vi "VIH HelpGen - Write HTML File - Menu - VI Table.vi"(4 "Show Item Icons":bool, 5 "HTML Folder":path, 6 "Items":T1, 7 "Image Folder":path, 8 "error in":errorcluster, 9 "Table Templates":T2, 10 "HTML in":string, 11 "Menu Path":path) -> (0 "error out":errorcluster, 2 "HTML out":string, 3 "dup Menu Path":path)   [LabVIEW 2014]
doc: "::: VI Helpeks :::\nCopyright (c) 2000-2026 Konstantin Shifershteyn. All rights reserved."
uses:
  VIH HelpGen Typedef - Table Templates Cluster - Menu Help.ctl
  VIH HelpGen Typedef - Enum - Description Mode.ctl
panel:
  # "VI Helpeks\nCopyright (c) 2012-2026 Konstantin Shifershteyn"
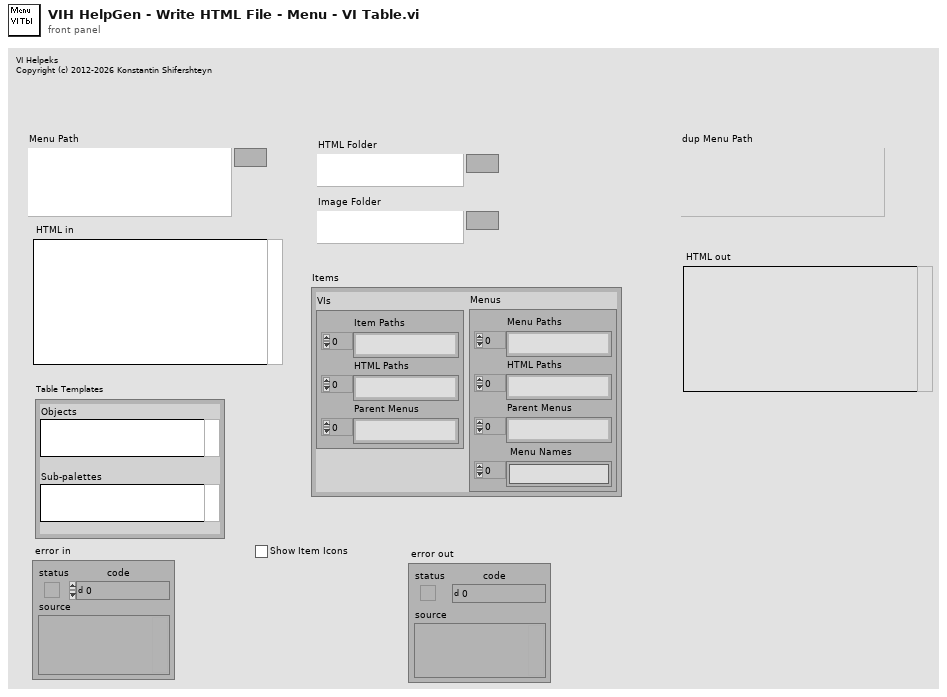
[diagram p1: front panel]
types:
  T1 = cluster{"VIs":cluster{"Item Paths":path[], "HTML Paths":path[], "Parent Menus":path[]}, "Menus":cluster{"Menu Paths":path[], "HTML Paths":path[], "Parent Menus":path[], " Menu Names":string[]}}
  T2 = typedef "VIH HelpGen Typedef - Table Templates Cluster - Menu Help.ctl" = cluster{"Objects":string, "Sub-palettes":string}
  T3 = typedef "VIH HelpGen Typedef - Palette - Item Info Cluster.ctl" = cluster{"Item Type":T4, "Item Name":string, "Item File":path, "Parent palette":path, "Not found":bool}
  T4 = typedef "VIH HelpGen Typedef - Palette - Item Type Enum.ctl" = enum32{"<Invalid>", "<unknown>", "VI", "Menu", "LV Func", "Express VI", "Poly VI", "CTL", "HTML"}
  T5 = cluster{"Item Paths":path[], "HTML Paths":path[], "Parent Menus":path[]}
  T6 = typedef "VIH HelpGen Typedef - Enum - Description Mode.ctl" = enum16{"Default", "Description", "Description1", "Description2", "Custom", "None"}
  T7 = typedef "imagedata.ctl" = cluster{"image type":i32, "image depth":i32, "image":u8[], "mask":u8[], "colors":u32[], "Rectangle":cluster{"left":i16, "top":i16, "right":i16, "bottom":i16}}
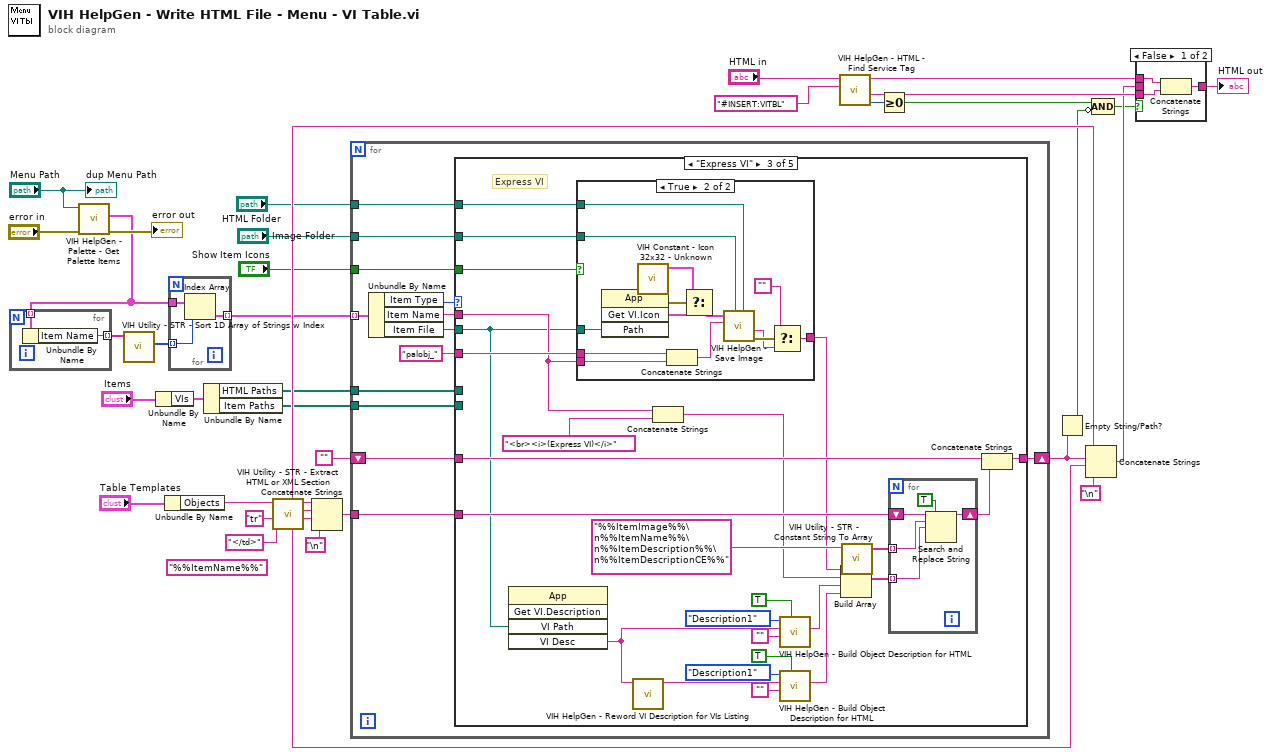
[diagram p0: block diagram]
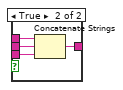
[diagram p2: hidden frame]
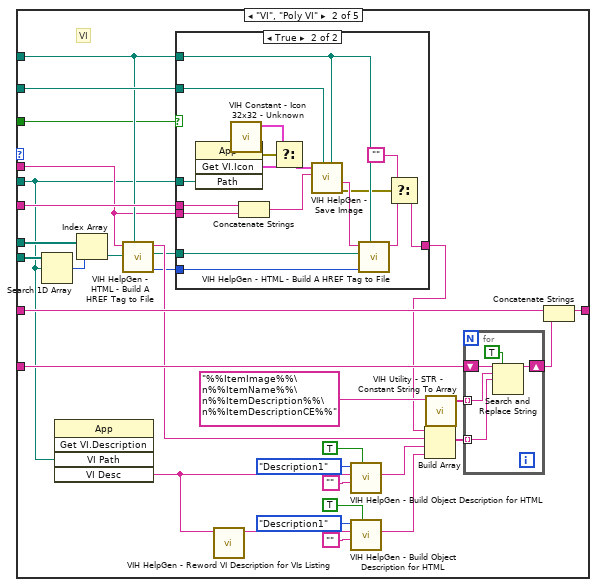
[diagram p4: hidden frame]
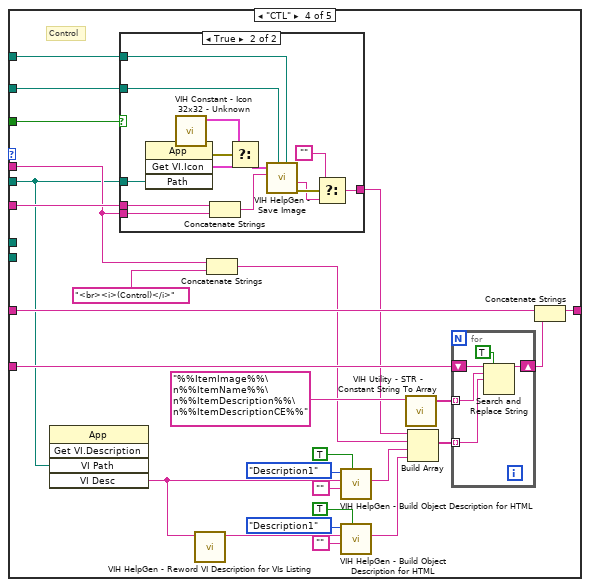
[diagram p7: hidden frame]
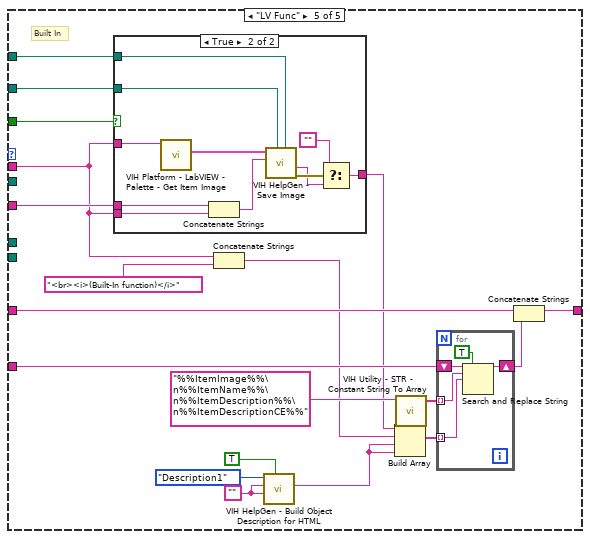
[diagram p9: hidden frame]
diagram:
  (unwired) "%%ItemName%%"
  n1 = call "VIH HelpGen - Palette - Get Palette Items.vi"("error in"="error in", "Palette Path"="Menu Path") -> ("error out"=→"error out":errorcluster, "Items Array"=w1:T3[])  [unwired: 7 in, 1 out]
  n2 = for {
    tunnel: [w40] -> w7 mode=indexing
    tunnel: w1 -> [w39] mode=indexing
    n3 = Unbundle By Name(w39) -> ("Item Name"=w40:string)
  }
  n4 = call "VIH Utility - STR - Sort 1D Array of Strings w Index.vi"("Array in"=w7) -> ("Index array"=w6:i32[])  [unwired: 7 in, 3 out]
  n5 = Unbundle By Name("Items") -> ("VIs"=w10:T5)
  n6 = Unbundle By Name("Table Templates") -> ("Objects"=w21:string)
  n7 = for {
    tunnel: w1 -> [w43]
    tunnel: w6 -> [w42] mode=indexing
    tunnel: [w41] -> w5 mode=indexing
    n8 = Index Array(array=w43, index=w42) -> (element=w41:T3)
  }
  n9 = Unbundle By Name(w10) -> ("HTML Paths"=w18:path[], "Item Paths"=w19:path[])
  n10 = call "VIH Utility - STR - Extract HTML or XML Section.vi"("Contain (opt)"="</td>", "Section name"="tr", "HTML in"=w21) -> ("end"=w30:string, "body"=w31:string, "start"=w32:string, "after"=w24:string, "before"=w25:string)  [unwired: 4 in]
  n11 = Concatenate Strings(w32, w31, w30, "\n") -> (w27:string)
  n12 = for {
    tunnel: w5 -> [w56] mode=indexing
    shift-right: [w50] -> w16
    shift-left: "" -> [w51]
    tunnel: w27 -> [w54]
    tunnel: w19 -> [w49]
    tunnel: w18 -> [w48]
    tunnel: "HTML Folder" -> [w47]
    tunnel: "Image Folder" -> [w46]
    tunnel: "Show Item Icons" -> [w44]
    n13 = Unbundle By Name(w56) -> ("Item Type"=w55:T4, "Item Name"=w53:string, "Item File"=w52:path)
    n14 = case shown="\"Express VI\"" w55 {
      tunnel: w54 -> [_ w85 w133 w178 w216]
      tunnel: w53 -> [_ w68 w119 w164 w202]
      tunnel: w52 -> [_ w65 w117 w162 _]
      tunnel: w51 -> [w57 w84 w132 w177 w215]
      tunnel: [w57 w83 w131 w176 w214] -> w50
      tunnel: w49 -> [_ w81 _ _ _]
      tunnel: w48 -> [_ w80 _ _ _]
      tunnel: w47 -> [_ w72 w127 w172 w210]
      tunnel: w46 -> [_ w78 w126 w171 w209]
      tunnel: "palobj_" -> [_ w77 w125 w170 w208]
      tunnel: w44 -> [_ w66 w118 w163 w203]
      frame "<Invalid>", "<unknown>", "Menu", "HTML" {
        # "Submenu, Empty"
      }
      frame "VI", "Poly VI" {
        # "VI"
        n15 = Search 1D Array(1D array=w81, element=w65) -> (index of element=w79:i32)  [unwired: 1 in]
        n16 = invoke class="App" method="Get VI.Description"("VI Path"=w65) -> ("VI Desc"=w59:string)  [unwired: 4 in, 4 out]
        n17 = Index Array(array=w80, index=w79) -> (element=w76:path)
        n18 = call "VIH HelpGen - HTML - Build A HREF Tag to File.vi"("HTML Folder"=w72, "Referenced HTML File"=w76, "Name"=w68) -> ("file status out"=w73:enum16{"unknown", "good", "bad"}, "dup Referenced HTML File"=w74:path, "HTML out"=w75:string)  [unwired: 6 in]
        n19 = case shown="True" w66 {
          tunnel: w78 -> [_ w105]
          tunnel: w77 -> [_ w103]
          tunnel: w74 -> [_ w102]
          tunnel: w73 -> [_ w101]
          tunnel: w72 -> [_ w100]
          tunnel: w68 -> [_ w98]
          tunnel: [_ w94] -> w67
          tunnel: w65 -> [_ w93]
          frame False {
          }
          frame True {
            n20 = invoke class="App" method="Get VI.Icon"("Path"=w93) -> (error out=w92:errorcluster, "Get VI.Icon"=w91:T7)  [unwired: 3 in, 2 out]
            n21 = call "VIH Constant - Icon 32x32 - Unknown.vi"() -> ("image data"=w89:T7)  [unwired: 11 in]
            n22 = Concatenate Strings(w103, w98) -> (w104:string)
            n23 = Select(t=w89, s=w92, f=w91) -> (s? t:f=w90:T7)
            n24 = call "VIH HelpGen - Save Image.vi"("HTML Folder"=w100, "Image Folder"=w105, "Image Filename"=w104, "image data"=w90) -> ("error out"=w96:errorcluster, "HTML tag"=w99:string)  [unwired: 5 in, 1 out]
            n25 = call "VIH HelpGen - HTML - Build A HREF Tag to File.vi"("HTML Folder"=w100, "file status"=w101, "Referenced HTML File"=w102, "Name"=w99) -> ("HTML out"=w95:string)  [unwired: 5 in, 2 out]
            n26 = Select(t="", s=w96, f=w95) -> (s? t:f=w94:string)
          }
        }
        n27 = call "VIH HelpGen - Reword VI Description for VIs Listing.vi"("String in"=w59) -> ("String out"=w63:string)  [unwired: 10 in]
        n28 = call "VIH HelpGen - Build Object Description for HTML.vi"("Ena \"No Description\" message (F)"=TRUE, "Custom Description"="", "Default Description"=w59, "DscrMode"=VIH_HelpGen_Typedef_-_Enum_-_Description_Mode."Description1") -> ("Description HTML out"=w58:string)  [unwired: 6 in, 1 out]
        n29 = call "VIH HelpGen - Build Object Description for HTML.vi"("Ena \"No Description\" message (F)"=TRUE, "Custom Description"="", "Default Description"=w63, "DscrMode"=VIH_HelpGen_Typedef_-_Enum_-_Description_Mode."Description1") -> ("Description HTML out"=w64:string)  [unwired: 6 in, 1 out]
        n30 = Build Array(w67, w75, w58, w64) -> (w86:string[])
        n31 = call "VIH Utility - STR - Constant String To Array.vi"("String in"="%%ItemImage%%\n%%ItemName%%\n%%ItemDescription%%\n%%ItemDescriptionCE%%") -> ("Array out"=w87:string[])  [unwired: 10 in]
        n32 = for {
          shift-right: [w109] -> w82
          shift-left: w85 -> [w110]
          tunnel: w87 -> [w107] mode=indexing
          tunnel: w86 -> [w106] mode=indexing
          n33 = Search and Replace String(replace all?=TRUE, input string=w110, search string=w107, replace string=w106) -> (result string=w109:string)  [unwired: 4 in, 3 out]
        }
        n34 = Concatenate Strings(w84, w82) -> (w83:string)
      }
      frame "Express VI" {
        # "Express VI"
        n35 = invoke class="App" method="Get VI.Description"("VI Path"=w117) -> ("VI Desc"=w112:string)  [unwired: 4 in, 4 out]
        n36 = case shown="True" w118 {
          tunnel: w127 -> [_ w149]
          tunnel: w126 -> [_ w148]
          tunnel: w125 -> [_ w147]
          tunnel: [_ w142] -> w124
          tunnel: w119 -> [_ w146]
          tunnel: w117 -> [_ w141]
          frame False {
          }
          frame True {
            n37 = invoke class="App" method="Get VI.Icon"("Path"=w141) -> (error out=w140:errorcluster, "Get VI.Icon"=w139:T7)  [unwired: 3 in, 2 out]
            n38 = call "VIH Constant - Icon 32x32 - Unknown.vi"() -> ("image data"=w137:T7)  [unwired: 11 in]
            n39 = Concatenate Strings(w147, w146) -> (w150:string)
            n40 = Select(t=w137, s=w140, f=w139) -> (s? t:f=w138:T7)
            n41 = call "VIH HelpGen - Save Image.vi"("HTML Folder"=w149, "Image Folder"=w148, "Image Filename"=w150, "image data"=w138) -> ("error out"=w144:errorcluster, "HTML tag"=w143:string)  [unwired: 5 in, 1 out]
            n42 = Select(t="", s=w144, f=w143) -> (s? t:f=w142:string)
          }
        }
        n43 = call "VIH HelpGen - Reword VI Description for VIs Listing.vi"("String in"=w112) -> ("String out"=w116:string)  [unwired: 10 in]
        n44 = Concatenate Strings(w119, "<br><i>(Express VI)</i>" ("string")) -> (w129:string)
        n45 = call "VIH HelpGen - Build Object Description for HTML.vi"("Ena \"No Description\" message (F)"=TRUE, "Custom Description"="", "Default Description"=w112, "DscrMode"=VIH_HelpGen_Typedef_-_Enum_-_Description_Mode."Description1") -> ("Description HTML out"=w111:string)  [unwired: 6 in, 1 out]
        n46 = call "VIH HelpGen - Build Object Description for HTML.vi"("Ena \"No Description\" message (F)"=TRUE, "Custom Description"="", "Default Description"=w116, "DscrMode"=VIH_HelpGen_Typedef_-_Enum_-_Description_Mode."Description1") -> ("Description HTML out"=w120:string)  [unwired: 6 in, 1 out]
        n47 = Build Array(w124, w129, w111, w120) -> (w134:string[])
        n48 = call "VIH Utility - STR - Constant String To Array.vi"("String in"="%%ItemImage%%\n%%ItemName%%\n%%ItemDescription%%\n%%ItemDescriptionCE%%") -> ("Array out"=w135:string[])  [unwired: 10 in]
        n49 = for {
          shift-right: [w154] -> w130
          shift-left: w133 -> [w155]
          tunnel: w135 -> [w152] mode=indexing
          tunnel: w134 -> [w151] mode=indexing
          n50 = Search and Replace String(replace all?=TRUE, input string=w155, search string=w152, replace string=w151) -> (result string=w154:string)  [unwired: 4 in, 3 out]
        }
        n51 = Concatenate Strings(w132, w130) -> (w131:string)
      }
      frame "CTL" {
        # "Control"
        n52 = invoke class="App" method="Get VI.Description"("VI Path"=w162) -> ("VI Desc"=w157:string)  [unwired: 4 in, 4 out]
        n53 = case shown="True" w163 {
          tunnel: w172 -> [_ w194]
          tunnel: w171 -> [_ w193]
          tunnel: w170 -> [_ w192]
          tunnel: [_ w187] -> w169
          tunnel: w164 -> [_ w191]
          tunnel: w162 -> [_ w186]
          frame False {
          }
          frame True {
            n54 = invoke class="App" method="Get VI.Icon"("Path"=w186) -> (error out=w185:errorcluster, "Get VI.Icon"=w184:T7)  [unwired: 3 in, 2 out]
            n55 = call "VIH Constant - Icon 32x32 - Unknown.vi"() -> ("image data"=w183:T7)  [unwired: 11 in]
            n56 = Concatenate Strings(w192, w191) -> (w195:string)
            n57 = Select(t=w183, s=w185, f=w184) -> (s? t:f=w182:T7)
            n58 = call "VIH HelpGen - Save Image.vi"("HTML Folder"=w194, "Image Folder"=w193, "Image Filename"=w195, "image data"=w182) -> ("error out"=w189:errorcluster, "HTML tag"=w188:string)  [unwired: 5 in, 1 out]
            n59 = Select(t="", s=w189, f=w188) -> (s? t:f=w187:string)
          }
        }
        n60 = call "VIH HelpGen - Reword VI Description for VIs Listing.vi"("String in"=w157) -> ("String out"=w161:string)  [unwired: 10 in]
        n61 = Concatenate Strings(w164, "<br><i>(Control)</i>" ("string")) -> (w174:string)
        n62 = call "VIH HelpGen - Build Object Description for HTML.vi"("Ena \"No Description\" message (F)"=TRUE, "Custom Description"="", "Default Description"=w157, "DscrMode"=VIH_HelpGen_Typedef_-_Enum_-_Description_Mode."Description1") -> ("Description HTML out"=w156:string)  [unwired: 6 in, 1 out]
        n63 = call "VIH HelpGen - Build Object Description for HTML.vi"("Ena \"No Description\" message (F)"=TRUE, "Custom Description"="", "Default Description"=w161, "DscrMode"=VIH_HelpGen_Typedef_-_Enum_-_Description_Mode."Description1") -> ("Description HTML out"=w165:string)  [unwired: 6 in, 1 out]
        n64 = call "VIH Utility - STR - Constant String To Array.vi"("String in"="%%ItemImage%%\n%%ItemName%%\n%%ItemDescription%%\n%%ItemDescriptionCE%%") -> ("Array out"=w180:string[])  [unwired: 10 in]
        n65 = Build Array(w169, w174, w156, w165) -> (w179:string[])
        n66 = for {
          shift-right: [w199] -> w175
          shift-left: w178 -> [w200]
          tunnel: w180 -> [w197] mode=indexing
          tunnel: w179 -> [w196] mode=indexing
          n67 = Search and Replace String(replace all?=TRUE, input string=w200, search string=w197, replace string=w196) -> (result string=w199:string)  [unwired: 4 in, 3 out]
        }
        n68 = Concatenate Strings(w177, w175) -> (w176:string)
      }
      frame "LV Func" {
        w204 = ""
        # "Built In"
        n69 = case shown="True" w203 {
          tunnel: w210 -> [_ w229]
          tunnel: w209 -> [_ w228]
          tunnel: w202 -> [_ w227]
          tunnel: w208 -> [_ w226]
          tunnel: [_ w223] -> w207
          tunnel: w202 -> [_ w221]
          frame False {
          }
          frame True {
            n70 = call "VIH Platform - LabVIEW - Palette - Get Item Image.vi"("Palette Item Name"=w221) -> ("Palette Item Icon"=w220:T7)  [unwired: 8 in, 2 out]
            n71 = Concatenate Strings(w226, w227) -> (w230:string)
            n72 = call "VIH HelpGen - Save Image.vi"("HTML Folder"=w229, "Image Folder"=w228, "Image Filename"=w230, "image data"=w220) -> ("error out"=w225:errorcluster, "HTML tag"=w224:string)  [unwired: 5 in, 1 out]
            n73 = Select(t="", s=w225, f=w224) -> (s? t:f=w223:string)
          }
        }
        n74 = Concatenate Strings(w202, "<br><i>(Built-In function)</i>" ("string")) -> (w212:string)
        n75 = call "VIH HelpGen - Build Object Description for HTML.vi"("Ena \"No Description\" message (F)"=TRUE, "Custom Description"=w204, "Default Description"=w204, "DscrMode"=VIH_HelpGen_Typedef_-_Enum_-_Description_Mode."Description1") -> ("Description HTML out"=w201:string)  [unwired: 6 in, 1 out]
        n76 = Build Array(w207, w212, w201, w201) -> (w217:string[])
        n77 = call "VIH Utility - STR - Constant String To Array.vi"("String in"="%%ItemImage%%\n%%ItemName%%\n%%ItemDescription%%\n%%ItemDescriptionCE%%") -> ("Array out"=w218:string[])  [unwired: 10 in]
        n78 = for {
          shift-right: [w234] -> w213
          shift-left: w216 -> [w235]
          tunnel: w218 -> [w232] mode=indexing
          tunnel: w217 -> [w231] mode=indexing
          n79 = Search and Replace String(replace all?=TRUE, input string=w235, search string=w232, replace string=w231) -> (result string=w234:string)  [unwired: 4 in, 3 out]
        }
        n80 = Concatenate Strings(w215, w213) -> (w214:string)
      }
    }
  }
  n81 = call "VIH HelpGen - HTML - Find Service Tag.vi"("Tag name"="#INSERT:VITBL", "HTML in"="HTML in") -> ("Offset out"=w15:i32, "After"=w36:string, "Before"=w37:string)  [unwired: 6 in, 1 out]
  n82 = Greater Or Equal To 0?(x=w15) -> (x >= 0?=w14:bool)
  n83 = Empty String/Path?(string/path=w16) -> (empty?=w13:bool)
  n84 = Concatenate Strings(w25, w16, w24, "\n") -> (w23:string)
  n85 = Compound Arithmetic op=AND(w14, invert w13) -> (w12:bool)
  n86 = case shown="False" w12 {
    tunnel: w23 -> [_ w242]
    tunnel: [w236 w241] -> w26
    tunnel: w37 -> [w238 w240]
    tunnel: w36 -> [w237 w239]
    frame False {
      n87 = Concatenate Strings(w238, w237) -> (w236:string)
    }
    frame True {
      n88 = Concatenate Strings(w240, w242, w239) -> (w241:string)
    }
  }
  "HTML out" <- w26
  "dup Menu Path" <- "Menu Path"
